vi "Select Component.vi"(7 "Disable Others?":T1, 8 "error in (no error)":errorcluster, 10 "Component":string, 11 "Camera in":refnum<class "Camera.lvclass">) -> (0 "error out":errorcluster, 3 "Camera":refnum<class "Camera.lvclass">)   [LabVIEW 2020, in "Camera.lvclass"]
uses:
  Camera.lvclass
  Component Selection Mode.ctl
  Camera.lvclass/Camera.ctl
  bin/gindustrialcam_32-1.dll
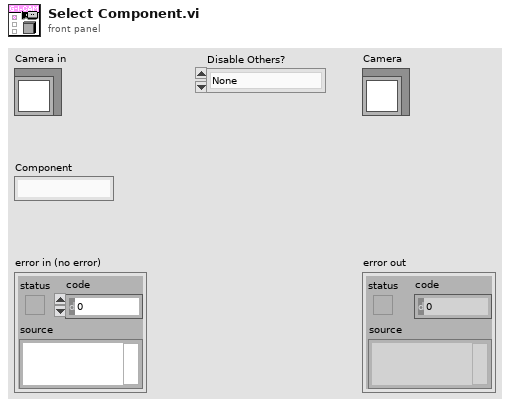
[diagram p1: front panel]
types:
  T1 = typedef "Camera.lvclass/Component Selection Mode.ctl" = enum8{"None", "Enable", "Disable", "Exclusive Enable", "Enable All"}
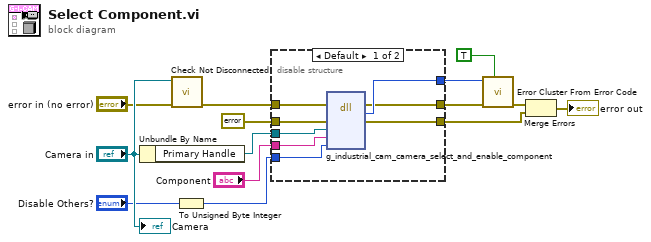
[diagram p0: block diagram]
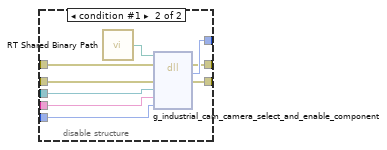
[diagram p2: hidden frame]
diagram:
  n1 = Unbundle By Name("Camera in") -> ("Primary Handle"=w9:refnum<data-value>)
  n2 = call "Check Not Disconnected.vi"("error in (no error)"="error in (no error)", "Camera in"="Camera in") -> ("error out"=w10:errorcluster)  [unwired: 9 in]
  n3 = To Unsigned Byte Integer(number="Disable Others?") -> (unsigned 8bit integer=w1:u8)
  n4 = disable-structure shown="Default" {
    disable-tunnel: w10 -> [w22 w31]
    disable-tunnel: w9 -> [w21 w30]
    disable-tunnel: errorcluster {"status"=FALSE, "code"=0, "source"=""} ("error constant") -> [w20 w29]
    disable-tunnel: [w19 w28] -> w6
    disable-tunnel: [w18 w27] -> w4
    disable-tunnel: [w17 w26] -> w3
    disable-tunnel: "Component" -> [w16 w25]
    disable-tunnel: w1 -> [w15 w24]
    frame condition #0 (active) {
      n5 = dll-call lib="C:/serenial/lib/g-industrial-camera/LabVIEW/g_industrial_cam/bin/gindustrialcam_*-1.*" fn="g_industrial_cam_camera_select_and_enable_component"(error in=w22, "err"=w20, "edvr"=w21, "component"=w16, "selection_mode"=w15) -> (error out=w17:errorcluster, "Mg_Error"=w18:i32, "err"=w19:errorcluster)  [unwired: 5 in, 1 out]
    }
    frame condition #1 {
      n6 = call "RT Shared Binary Path.vi"() -> ("Path"=w23:path)
      n7 = dll-call lib="C:/serenial/lib/g-industrial-camera/LabVIEW/g_industrial_cam/bin/gindustrialcam_*-1.*" fn="g_industrial_cam_camera_select_and_enable_component"(path in=w23, error in=w31, "err"=w29, "edvr"=w30, "component"=w25, "selection_mode"=w24) -> (error out=w26:errorcluster, "Mg_Error"=w27:i32, "err"=w28:errorcluster)  [unwired: 4 in, 1 out]
    }
  }
  n8 = call <vilib>:"Error Cluster From Error Code.vi"("show call chain? (False)"=TRUE, "error in (no error)"=w3, "error code (0)"=w4) -> ("error out"=w5:errorcluster)  [unwired: 6 in]
  n9 = Merge Errors(w5, w6) -> (→"error out":errorcluster)
  "Camera" <- "Camera in"
